vi "Alarm_Capture.vi"(7 "AlarmText in":string, 8 "error in (no error)":errorcluster, 9 "AlarmCode in":i32, 10 "CurrentState":T1, 11 "NextState":T1) -> (1 "AlarmText out":string, 2 "AlarmCode out":i32, 3 "NextFinal":T1, 4 "InAlarm":bool)   [LabVIEW 2018]
uses:
  07_QMH.vi/State.ctl
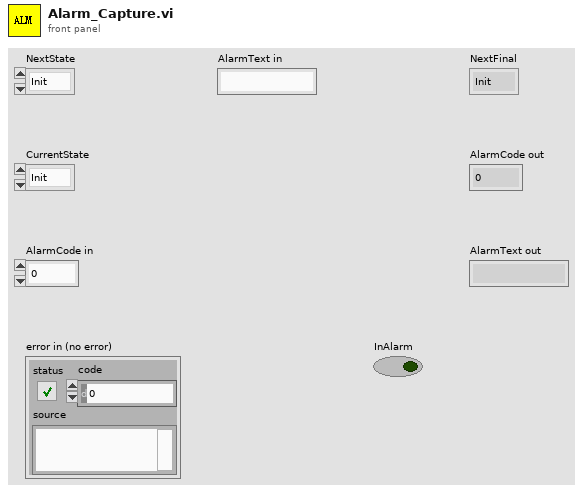
[diagram p1: front panel]
types:
  T1 = typedef "State.ctl" = enum16{"Init", "RequestPart", "WaitEntry", "WaitInPos", "WaitClamp", "Inspect", "Release", "WaitRelease", "WaitSort", "PushNG", "WaitPushExt", "WaitPushRet", "DeliverOK", "WaitExit", "WaitExitClear", "Done", "Error", "Stop", "Idle", "Pause", "Resume", "AlarmWait", "PurgeStart", "PurgeRun", "PurgePush", "PurgePushRet", "PurgeEnd"}
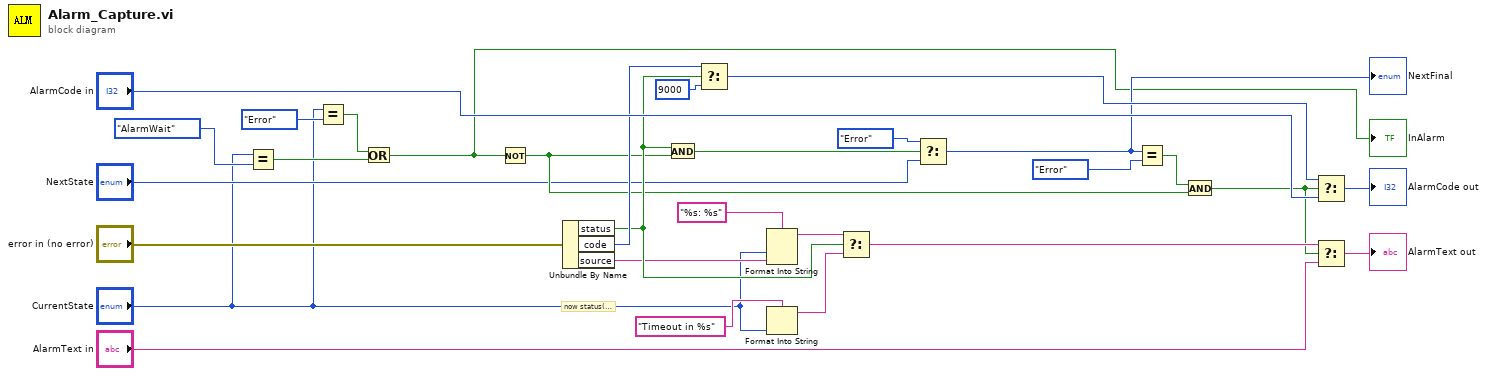
[diagram p0: block diagram]
diagram:
  # "now status(s r1)"
  n1 = Equal?(x="CurrentState", y=State."AlarmWait" ("Enum")) -> (x = y?=w5:bool)
  n2 = Equal?(x="CurrentState", y=State."Error" ("Enum")) -> (x = y?=w4:bool)
  n3 = Or(x=w4, y=w5) -> (x .or. y?=w6:bool)
  "InAlarm" <- w6
  n4 = Not(x=w6) -> (.not. x?=w11:bool)
  n5 = Unbundle By Name("error in (no error)") -> ("status"=w16:bool, "code"=w19:i32, "source"=w14:string)
  n6 = And(x=w16, y=w11) -> (x .and. y?=w7:bool)
  n7 = Select(t=w19, s=w16, f=9000) -> (s? t:f=w22:i32)
  n8 = Format Into String(format string="%s: %s", "CurrentState", w14) -> (resulting string=w17:string)  [unwired: 2 in, 1 out]
  n9 = Format Into String(format string="Timeout in %s", "CurrentState") -> (resulting string=w18:string)  [unwired: 2 in, 1 out]
  n10 = Select(t=w17, s=w16, f=w18) -> (s? t:f=w23:string)
  n11 = Select(t=State."Error" ("Enum"), s=w7, f="NextState") -> (s? t:f=w12:T1)
  "NextFinal" <- w12
  n12 = Equal?(x=w12, y=State."Error" ("Enum")) -> (x = y?=w10:bool)
  n13 = And(x=w10, y=w11) -> (x .and. y?=w21:bool)
  n14 = Select(t=w22, s=w21, f="AlarmCode in") -> (s? t:f=→"AlarmCode out":i32)
  n15 = Select(t=w23, s=w21, f="AlarmText in") -> (s? t:f=→"AlarmText out":string)
